vi "DAC Init Results.vi"(8 "error in":errorcluster, 9 "Log Details?":bool, 10 "tdms file":refnum<k34>, 11 "DAC FTCU in":refnum<class "DAC FTCU.lvclass">) -> (0 "error out":errorcluster, 2 "tdms file out":refnum<k34>)   [LabVIEW 2019, in "DAC.lvlib" / "DAC FTCU.lvclass"]
uses:
  DAC FTCU.lvclass
  DAC.lvclass
  C:/Users/wg/Documents/LV_Projects/test-stand/App/DAC/DAC.lvclass
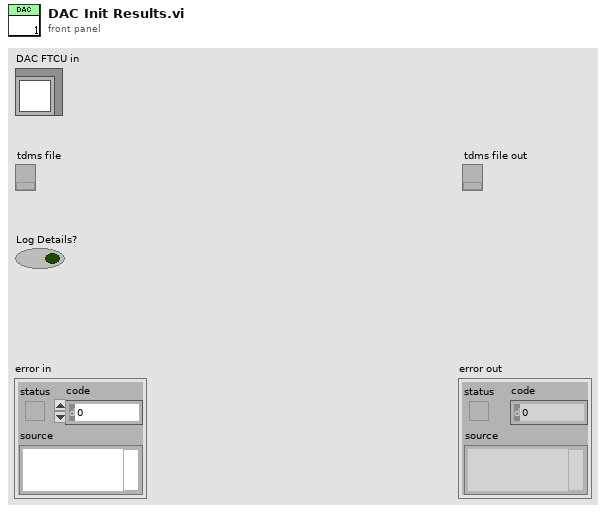
[diagram p1: front panel]
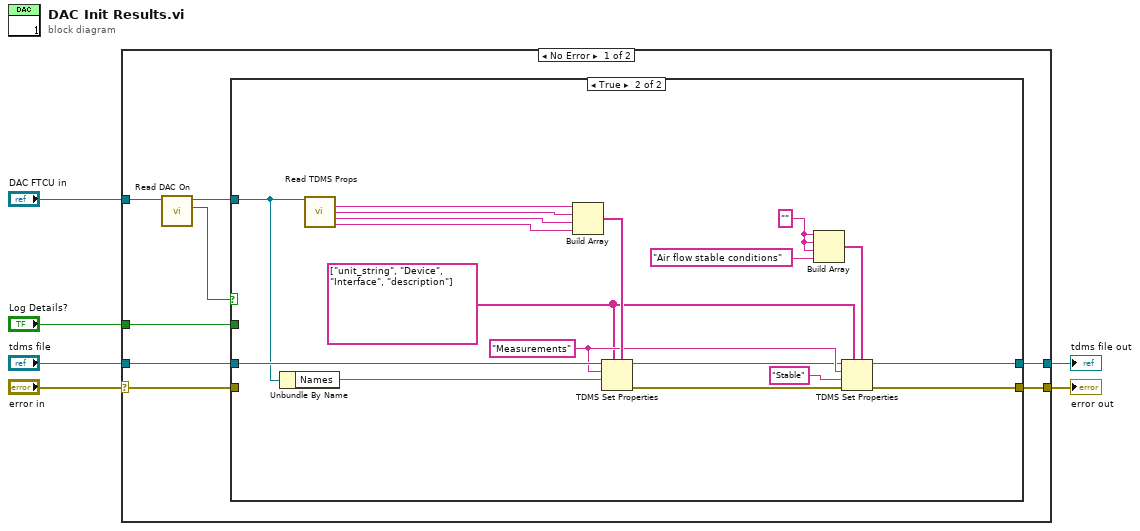
[diagram p0: block diagram]
diagram:
  n1 = case shown="No Error" "error in" {
    selector: "error in" -> [w9 w36]
    tunnel: [w12 w36] -> w3
    tunnel: "DAC FTCU in" -> [w11 _]
    tunnel: "tdms file" -> [w14 w35]
    tunnel: [w13 w35] -> w2
    tunnel: "Log Details?" -> [w7 _]
    frame No Error {
      n2 = call "Read DAC On.vi"("DAC in"=w11) -> ("DAC On"=w8:bool, "DAC out"=w10:refnum<class "DAC FTCU.lvclass">)  [unwired: 8 in, 1 out]
      n3 = case shown="True" w8 {
        tunnel: w14 -> [w16 w34]
        tunnel: [w16 w17] -> w13
        tunnel: [w15 w19] -> w12
        tunnel: w10 -> [_ w33]
        tunnel: w9 -> [w15 _]
        tunnel: w7 -> [_ _]
        frame False {
        }
        frame True {
          w26 = "" ("group name in (Untitled)")
          w23 = "Measurements" ("group name in (Untitled)")
          w22 = string[] ["unit_string", "Device", "Interface", "description"] ("property names")
          n4 = Unbundle By Name(w33) -> ("Names"=w24:string)
          n5 = call "Read TDMS Props.vi"("DAC in"=w33) -> ("Result Unit"=w31:string, "DAC Device"=w30:string, "DAC IO"=w29:string, "DAC Description"=w28:string)  [unwired: 10 in, 1 out]
          n6 = Build Array(w31, w30, w29, w28) -> (w32:string[])
          n7 = TDMS Set Properties(5:w32, 7:w22, 9:w24, 10:w23, 11:w34) -> (0:w20:errorcluster, 3:w18:refnum<k34>)  [unwired: 1 in, 2 out]
          n8 = Build Array(w26, w26, w26, "Air flow stable conditions" ("group name in (Untitled)")) -> (w27:string[])
          n9 = TDMS Set Properties(5:w27, 7:w22, 8:w20, 9:"Stable" ("delimiter"), 10:w23, 11:w18) -> (0:w19:errorcluster, 3:w17:refnum<k34>)  [unwired: 2 out]
        }
      }
    }
    frame Error {
    }
  }
  "error out" <- w3
  "tdms file out" <- w2
